vi "PrimaryProvider_CreateDummyObject.vi"(6 "error in":errorcluster, 9 "Wizard":T2) -> (0 "error out":errorcluster, 3 "Cancelled?":bool)   [LabVIEW 2023]
doc: "Use this template to create a wizard dialog."
uses:
  <resource>/Framework/Providers/API/ItemRef.ctl
panel:
  in  "Description":string
  in  "Selection":T1(radio)
  in  "Icon Color":u32(colorbox)=13631442
  in  "Operations":string="make\nsome\ndefaults"
  in  "Name":string="Swerve"
  in  "Cancel Button":bool
  in  "OK Button":bool
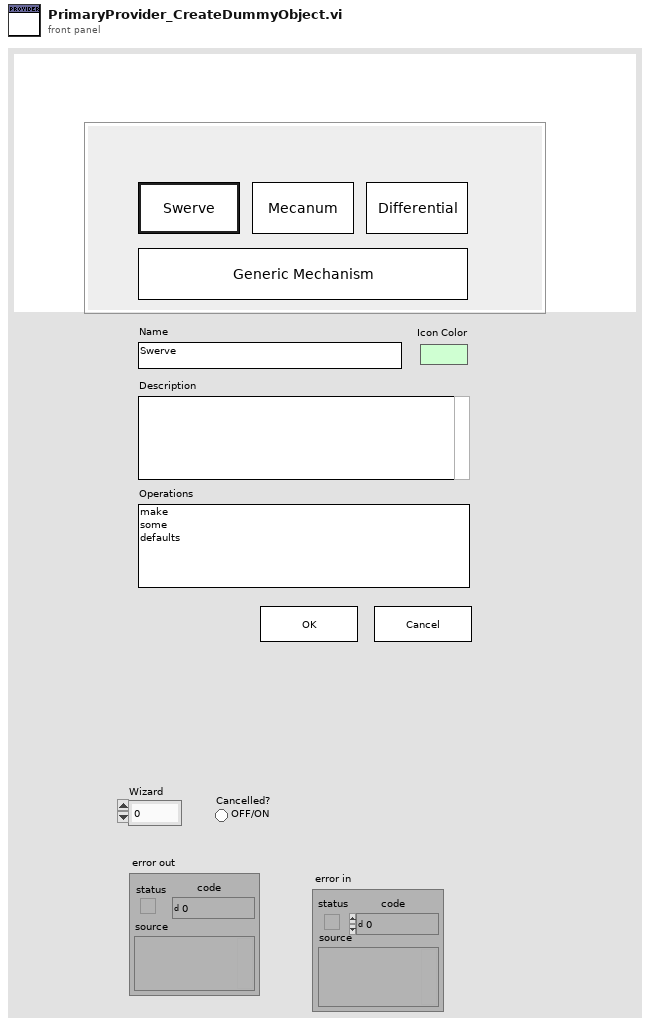
[diagram p1: front panel]
types:
  T1 = enum32{"Swerve ", "Mecanum", "Differential", "Generic"}
  T2 = typedef "ItemRef.ctl" = u64
  T3 = cluster{"Disabled":enum8{"Enabled", "Disabled", "Disabled and Grayed Out"}, "name":string, "ops":string, u32, "descr":string}[]
  T4 = cluster{"Disabled":enum8{"Enabled", "Disabled", "Disabled and Grayed Out"}, "name":string, "ops":string, u32, "descr":string}
  T5 = enum8{"Enabled", "Disabled", "Disabled and Grayed Out"}
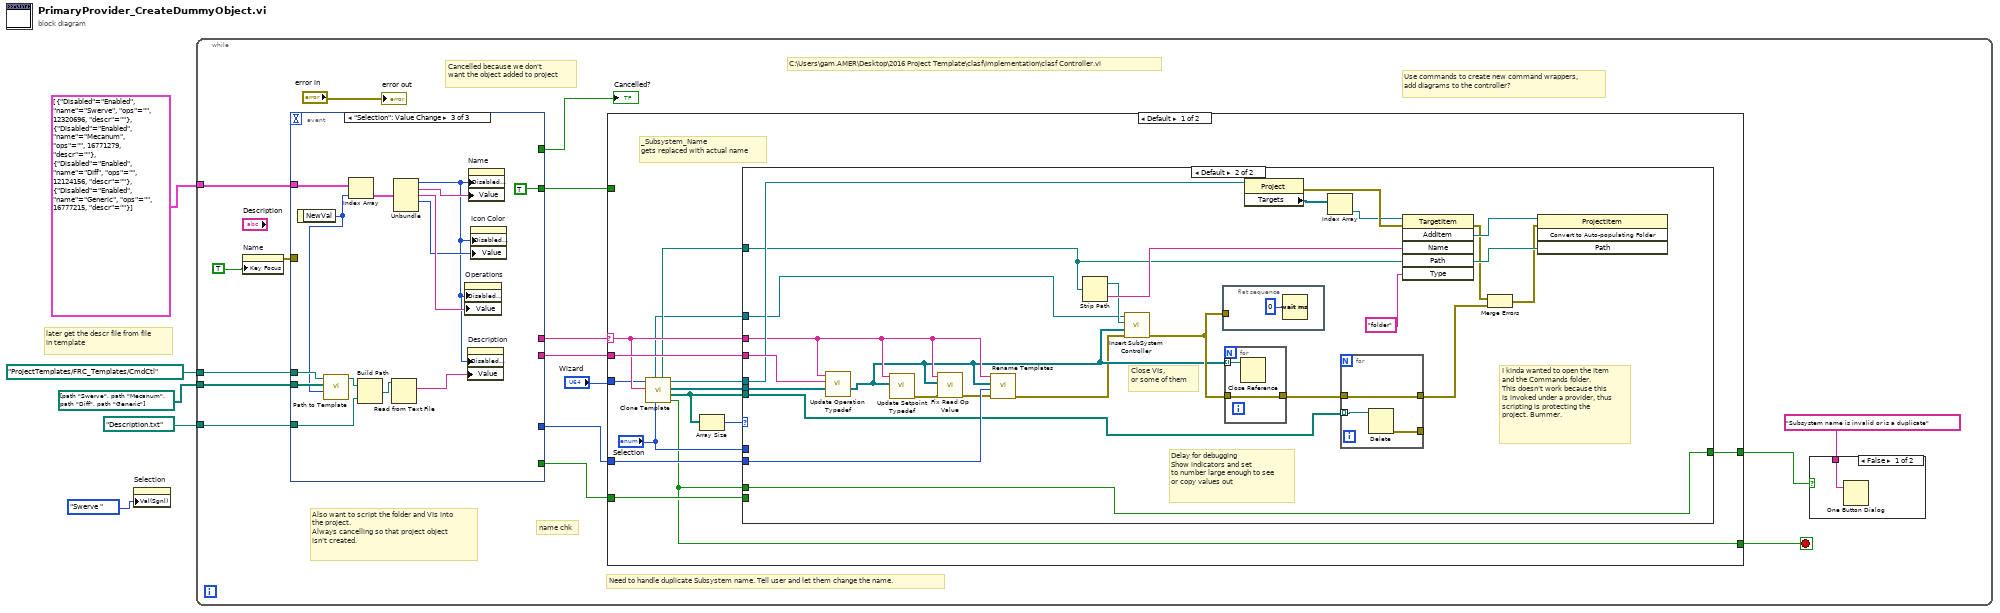
[diagram p0: block diagram]
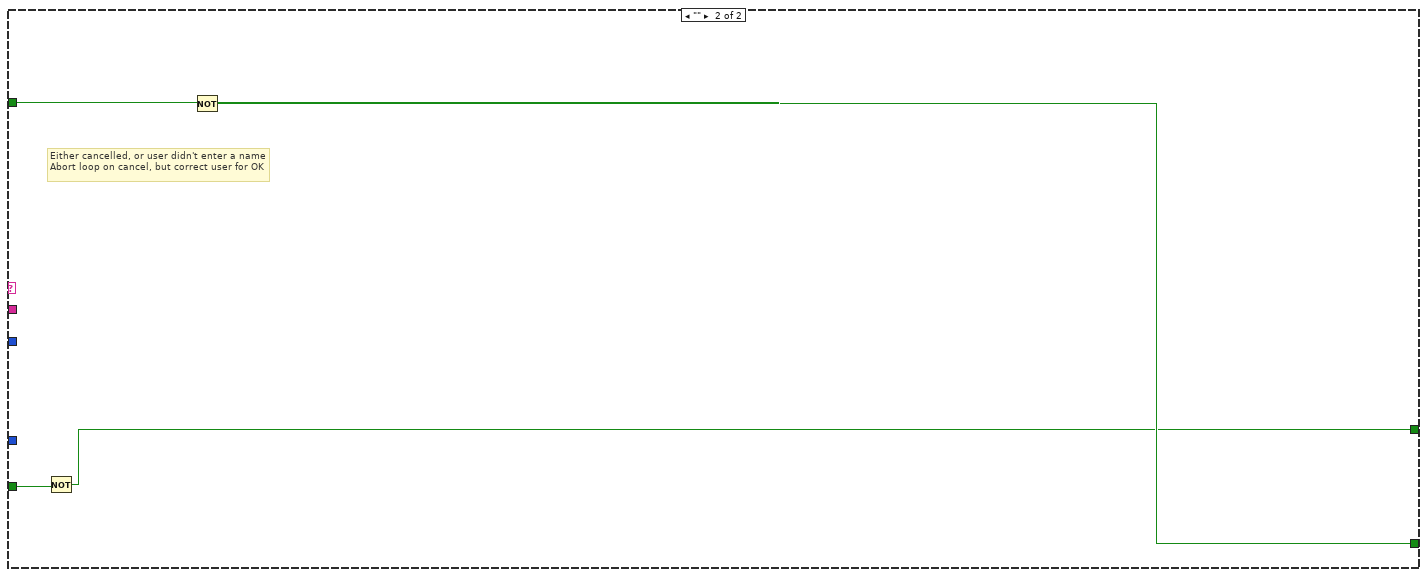
[diagram p3: hidden frame]
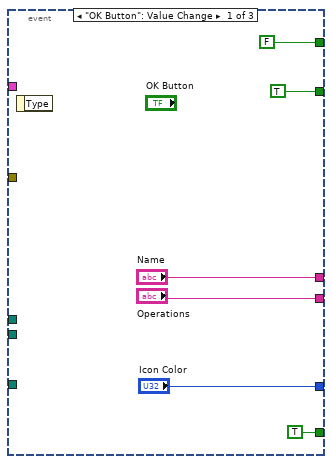
[diagram p5: hidden frame]
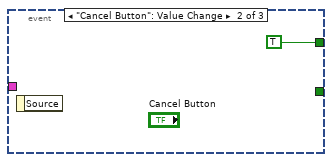
[diagram p6: hidden frame]
diagram:
  # "later get the descr file from file\nin template"
  n1 = property on="Selection" class="RadioBtnsControl (strict)"("Val(Sgnl)"=T1."Swerve " ("Value (Signaling)")) -> ()  [unwired: 2 in, 2 out]
  n2 = while {
    tunnel: T3 [{"Disabled"=enum."Enabled", "name"="Swerve", "ops"="", 12320696, "descr"=""}, {"Disabled"=enum."Enabled", "name"="Mecanum", "ops"="", 16771279, "descr"=""}, {"Disabled"=enum."Enabled", "name"="Diff", "ops"="", 12124156, "descr"=""}, {"Disabled"=enum."Enabled", "name"="Generic", "ops"="", 16777215, "descr"=""}] -> [w13]
    tunnel: path[] [path "Swerve", path "Mecanum", path "Diff", path "Generic"] -> [w8]
    tunnel: path "ProjectTemplates/FRC_Templates/CmdCtl" -> [w7]
    tunnel: path "Description.txt" ("name or relative path") -> [w6]
    stop <- w12 stop-if-true
    # "name chk"
    # "C:\\Users\\gam.AMER\\Desktop\\2016 Project Template\\clasf\\Implementation\\clasf Controller.vi"
    # "Use commands to create new command wrappers,\nadd diagrams to the controller?"
    # "Need to handle duplicate Subsystem name. Tell user and let them change the name."
    # "Cancelled because we don't\nwant the object added to project"
    # "Also want to script the folder and VIs into\nthe project.\nAlways cancelling so that project object\nisn't created."
    n3 = property on="Name" class="Str"("Key Focus"=TRUE) -> (error out=w18:errorcluster)  [unwired: 2 in, 1 out]
    n4 = event shown="[2] \"Selection\": Value Change" {
      selector: _ -> [_ _ _]
      dyn-events: _ -> [_ _ _]
      timeout: _ -> [_ _ _]
      tunnel: [FALSE ("Cancelled?") TRUE ("Cancelled?") _] -> w21
      tunnel: ["Name" _ _] -> w20
      tunnel: ["Operations" _ _] -> w19
      tunnel: w18 -> [_ _ _]
      tunnel: [TRUE ("Cancelled?") _ TRUE ("Cancelled?")] -> w16
      tunnel: ["Icon Color" _ _] -> w14
      tunnel: w13 -> [_ _ w94]
      tunnel: [TRUE ("Cancelled?") _ _] -> w10
      tunnel: w8 -> [_ _ w87]
      tunnel: w7 -> [_ _ w86]
      tunnel: w6 -> [_ _ w83]
      event "OK Button": Value Change {
        n5 = event-data() -> ()  [unwired: 1 in, 1 out]
      }
      event "Cancel Button": Value Change {
        n6 = event-data() -> ()  [unwired: 1 in, 1 out]
      }
      event "Selection": Value Change {
        n7 = event-data() -> ("NewVal"=w85:T1)  [unwired: 1 in]
        n8 = call <resource>:"Path to Template.vi"("Selector"=w85, "Array"=w87, "Path"=w86) -> ("resolved path"=w84:path)  [unwired: 8 in]
        n9 = Index Array(array=w94, index=w85) -> (element=w93:T4)
        n10 = Build Path(base path=w84, name or relative path=w83) -> (appended path=w82:path)
        n11 = Read from Text File(file (use dialog)=w82) -> (text=w81:string)  [unwired: 3 in, 3 out]
        n12 = Unbundle(w93) -> ("Disabled"=w88:T5, "name"=w91:string, "ops"=w92:string, w90:u32)  [unwired: 1 out]
        n13 = property on="Operations" class="Str"("DisabledEnum"=w88, "Value"=w92) -> ()  [unwired: 2 in, 2 out]
        n14 = property on="Description" class="Str"("DisabledEnum"=w88, "Value"=w81) -> ()  [unwired: 2 in, 2 out]
        n15 = property on="Name" class="Str"("DisabledEnum"=w88, "Value"=w91) -> ()  [unwired: 2 in, 2 out]
        n16 = property on="Icon Color" class="ColBox"("DisabledEnum"=w88, "Value"=w90) -> ()  [unwired: 2 in, 2 out]
      }
    }
    "Cancelled?" <- w21
    n17 = case shown="Default" w20 {
      selector: w20 -> [w34 _]
      tunnel: w19 -> [w35 _]
      tunnel: "Wizard" -> [w31 _]
      tunnel: [w24 w71] -> w12
      tunnel: w16 -> [_ w72]
      tunnel: w14 -> [w28 _]
      tunnel: [w26 w69] -> w11
      tunnel: w10 -> [w25 w70]
      frame Default {
        # "_Subsystem_Name\ngets replaced with actual name"
        n18 = call <resource>:"Clone Template.vi"("Selector"="Selection", "Subsystem Name"=w34, "Wizard"=w31) -> ("Success"=w24:bool, "Paths"=w33:path[], "VI Refs"=w36:refnum<vi>[], "Project Refnum"=w30:refnum<vi>, "Subsystem Path"=w32:path, "Application"=w29:refnum<vi>)  [unwired: 3 in]
        n19 = Array Size(array=w33) -> (size(s)=w23:i32)
        n20 = case shown="Default" w23 {
          tunnel: w36 -> [_ w62]
          tunnel: w35 -> [_ w61]
          tunnel: w34 -> [_ w53]
          tunnel: w33 -> [_ w40]
          tunnel: w32 -> [_ w51]
          tunnel: w30 -> [_ w56]
          tunnel: w29 -> [_ w41]
          tunnel: w28 -> [_ w54]
          tunnel: "Selection" -> [_ _]
          tunnel: [w37 w50] -> w26
          tunnel: w25 -> [_ _]
          tunnel: w24 -> [w37 w50]
          frame 0 {
          }
          frame Default {
            # "I kinda wanted to open the item\nand the Commands folder.\nThis doesn't work because this\nis invoked under a provider, thus\nscripting is protecting the\nproject. Bummer."
            # "Close VIs,\nor some of them"
            # "Delay for debugging\nShow indicators and set\nto number large enough to see\nor copy values out"
            n21 = call <resource>:"Update Operation Typedef.vi"("VI Refs"=w62, "Imm Cmd String"=w61, "Subsysten Name"=w53) -> ("VI Refs"=w52:refnum<vi>[])  [unwired: 7 in, 1 out]
            n22 = call <resource>:"Update Setpoint Typedef.vi"("VI Refs"=w52, "Subsystem Name"=w53) -> ("error out"=w39:errorcluster)  [unwired: 9 in]
            n23 = call <resource>:"Fix Read Op Value.vi"("error in (no error)"=w39, "VI Refs"=w52, "Subsystem Name"=w53) -> ("error in (no error) 2"=w38:errorcluster)  [unwired: 8 in]
            n24 = call <resource>:"Rename Templates.vi"("error in (no error)"=w38, "Icon Color"=w54, "VI Refs"=w52, "Subsystem Name"=w53) -> ("error out"=w42:errorcluster)  [unwired: 7 in]
            n25 = Strip Path(path=w51) -> (stripped path=w43:path, name=w60:string)
            n26 = call <resource>:"Insert SubSystem Controller.vi"("error in (no error)"=w42, "VI Refs"=w52, "Project Folder"=w43, "Application in"=w41) -> ("error out"=w55:errorcluster)  [unwired: 7 in]
            n27 = flat-sequence {
              tunnel: w55 -> [_]
              frame #0 {
                n28 = Wait (ms)(milliseconds to wait=u32 0) -> ()  [unwired: 1 out]
              }
            }
            n29 = for {
              tunnel: w55 -> [w64]
              tunnel: [w64] -> w57
              tunnel: w52 -> [w65] mode=indexing
              n30 = Close Reference(reference=w65) -> ()  [unwired: 1 in, 1 out]
            }
            n31 = property class="Project"(reference=w56) -> (error out=w58:errorcluster, "Targets"=w59:refnum<vi>[])  [unwired: 1 in, 1 out]
            n32 = Index Array(array=w59) -> (element=w49:refnum<vi>)  [unwired: 1 in]
            n33 = for {
              tunnel: w40 -> [w68] mode=indexing
              tunnel: w57 -> [w67]
              tunnel: [w67] -> w47
              tunnel: [w66] -> _
              n34 = Delete(path (use dialog)=w68) -> (error out=w66:errorcluster)  [unwired: 4 in, 2 out]
            }
            n35 = invoke class="TargetItem" method="AddItem"(reference=w49, error in=w58, "Name"=w60, "Path"=w51, "Type"="folder") -> (error out=w45:errorcluster, "AddItem"=w46:refnum<vi>)  [unwired: 1 in, 4 out]
            n36 = Merge Errors(w45, w47) -> (w44:errorcluster)
            n37 = invoke class="ProjectItem" method="Convert to Auto-populating Folder"(reference=w46, error in=w44, "Path"=w51) -> ()  [unwired: 1 in, 4 out]
          }
        }
      }
      frame "" {
        # "Either cancelled, or user didn't enter a name\nAbort loop on cancel, but correct user for OK"
        n38 = Not(x=w70) -> (.not. x?=w69:bool)
        n39 = Not(x=w72) -> (.not. x?=w71:bool)
      }
    }
    n40 = case shown="False" w11 {
      tunnel: "Subsystem name is invalid or is a duplicate" ("message") -> [w73 _]
      frame False {
        n41 = One Button Dialog(message=w73) -> ()  [unwired: 1 in, 1 out]
      }
      frame True {
      }
    }
    "error out" <- "error in"
  }
